vi "DUT_Connection_check.vi"(8 "error in":errorcluster, 9 "Enable":bool=TRUE, 11 "Text.Text Colors:BG Color":u32(colorbox)=16448250) -> (0 "error out":errorcluster, 1 "PASS":bool)   [LabVIEW 2021]
panel:
  out "Cancel 2":bool
  in  "Checkbox 3":bool
  in  "Checkbox 2":bool
  in  "Checkbox":bool
  in  "Continue":bool
  in  "Cancel":bool
  out "String":string
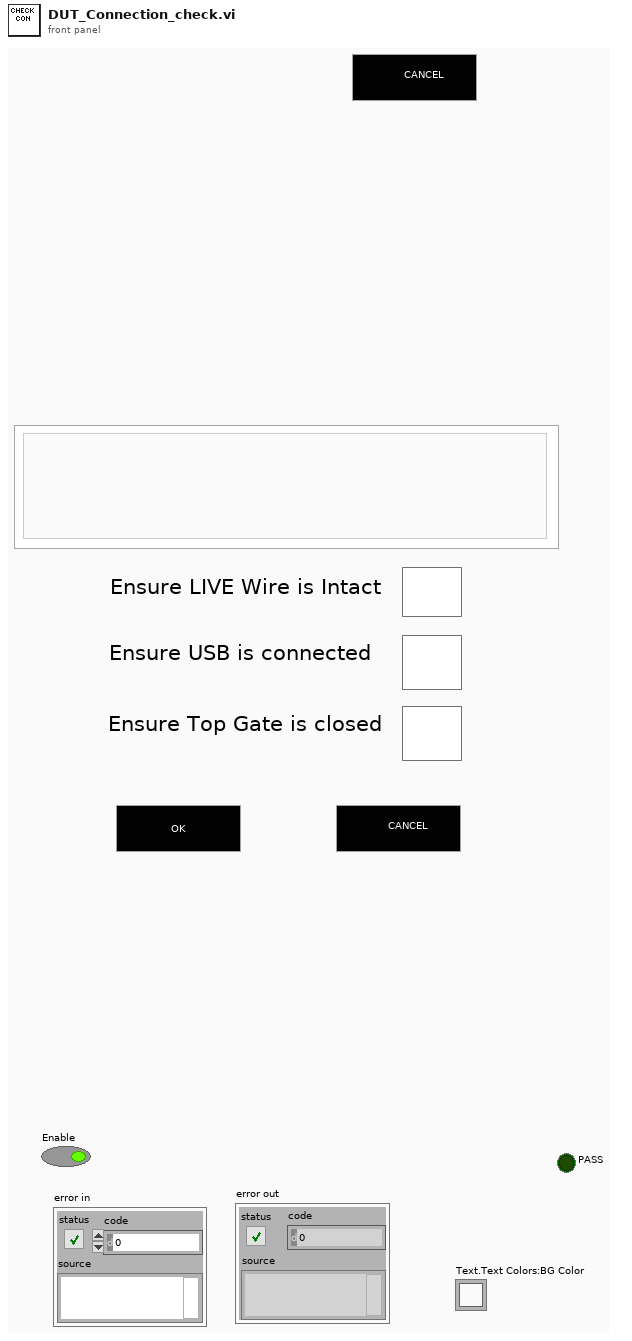
[diagram p1: front panel]
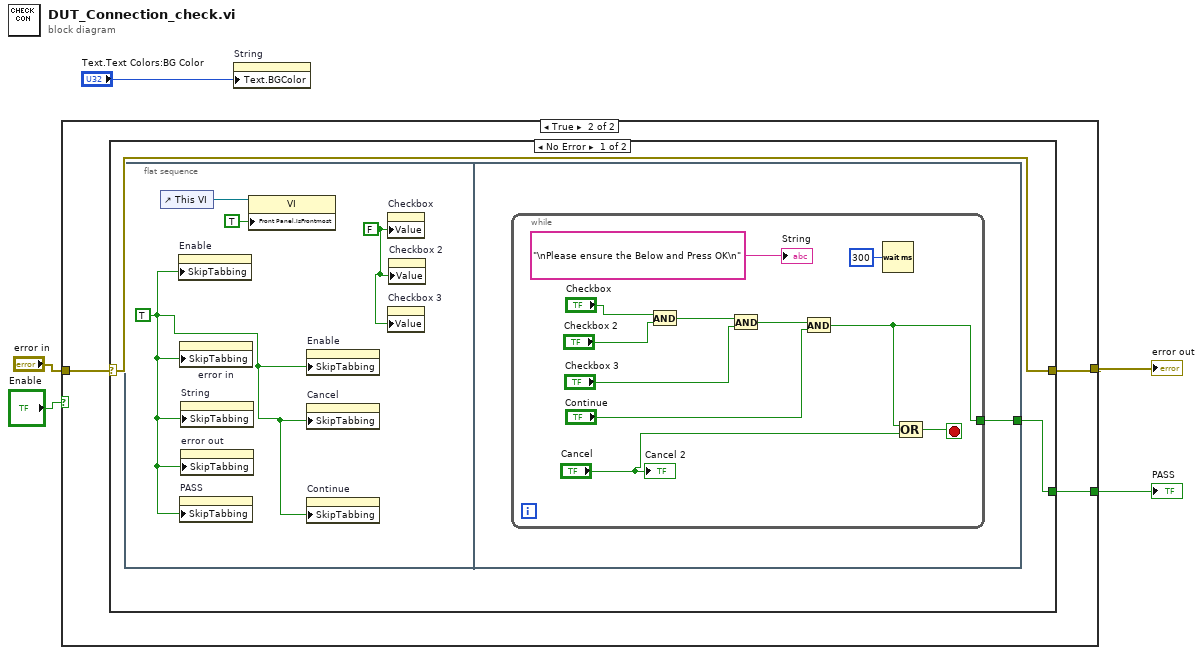
[diagram p0: block diagram]
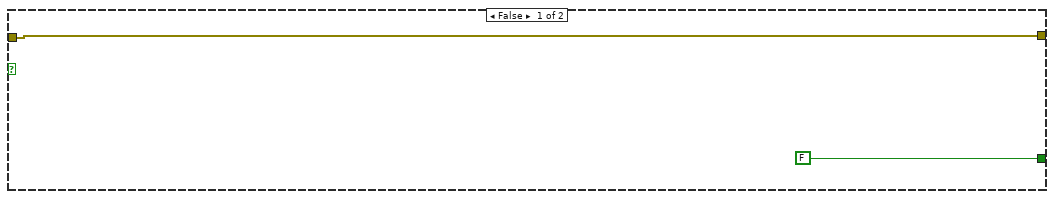
[diagram p2: hidden frame]
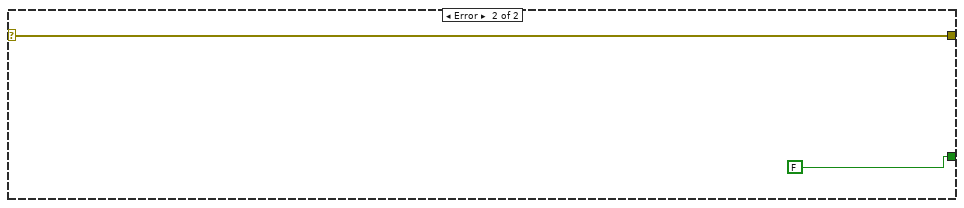
[diagram p3: hidden frame]
diagram:
  n1 = case shown="True" "Enable" {
    tunnel: "error in" -> [w7 w10]
    tunnel: [w7 w9] -> w4
    tunnel: [FALSE ("OK Button") w8] -> w2
    frame False {
    }
    frame True {
      n2 = case shown="No Error" w10 {
        selector: w10 -> [w12 w30]
        tunnel: [w12 w30] -> w9
        tunnel: [w11 FALSE ("OK Button")] -> w8
        frame No Error {
          n3 = flat-sequence {
            tunnel: [w17] -> w11
            frame #0 {
              w13 = FALSE ("Checkbox")
              w14 = TRUE ("Skip When Tabbing")
              n4 = control-ref of="This VI"() -> (w16:refnum<vi>)
              n5 = property on="Enable" class="Bool (strict)"("SkipTabbing"=w14) -> ()  [unwired: 2 in, 2 out]
              n6 = property on="error in" class="Clust (strict)"("SkipTabbing"=w14) -> ()  [unwired: 2 in, 2 out]
              n7 = property on="PASS" class="Bool (strict)"("SkipTabbing"=w14) -> ()  [unwired: 2 in, 2 out]
              n8 = property on="String" class="Str"("SkipTabbing"=w14) -> ()  [unwired: 2 in, 2 out]
              n9 = property on="error out" class="Clust (strict)"("SkipTabbing"=w14) -> ()  [unwired: 2 in, 2 out]
              n10 = property class="VI"(reference=w16, "Front Panel.IsFrontmost"=TRUE ("Front Panel Window:Is Frontmost")) -> ()  [unwired: 1 in, 2 out]
              n11 = property on="Enable" class="Bool (strict)"("SkipTabbing"=w14) -> ()  [unwired: 2 in, 2 out]
              n12 = property on="Cancel" class="Bool"("SkipTabbing"=w14) -> ()  [unwired: 2 in, 2 out]
              n13 = property on="Continue" class="Bool"("SkipTabbing"=w14) -> ()  [unwired: 2 in, 2 out]
              n14 = property on="Checkbox" class="Bool (strict)"("Value"=w13) -> ()  [unwired: 2 in, 2 out]
              n15 = property on="Checkbox 3" class="Bool (strict)"("Value"=w13) -> ()  [unwired: 2 in, 2 out]
              n16 = property on="Checkbox 2" class="Bool (strict)"("Value"=w13) -> ()  [unwired: 2 in, 2 out]
            }
            frame #1 {
              n17 = while {
                tunnel: [w20] -> w17
                stop <- w18 stop-if-true
                n18 = And(x="Checkbox", y="Checkbox 2") -> (x .and. y?=w24:bool)
                n19 = And(x=w24, y="Checkbox 3") -> (x .and. y?=w22:bool)
                n20 = And(x=w22, y="Continue") -> (x .and. y?=w20:bool)
                n21 = Wait (ms)(milliseconds to wait=u32 300) -> ()  [unwired: 1 out]
                n22 = Compound Arithmetic op=OR(w20, "Cancel") -> (w18:bool)
                "String" <- "\nPlease ensure the Below and Press OK\n" ("String")
                "Cancel 2" <- "Cancel"
              }
            }
          }
        }
        frame Error {
        }
      }
    }
  }
  "error out" <- w4
  "PASS" <- w2
  n23 = property on="String" class="Str"("Text.BGColor"="Text.Text Colors:BG Color") -> ()  [unwired: 2 in, 2 out]
